vi "Define_Indicies_Connect_Points_Subtracks-1.vi"(3 "error IN":errorcluster, 4 "[IN] Index of track with\n(problem displacement)":i32, 5 "[IN] Index of problem\ndisplacement inside track":i32, 6 "[IN] Track group":T1) -> (0 "error OUT":errorcluster, 1 "[OUT] Index of \nconnected dots\ninside the track":i32[](array[numeric]), 2 "[OUT] Index of connected\ntracks with problem dot":i32[](array[numeric]))   [LabVIEW 2017]
doc: "The subVI scans subtracks for defining connected with input problem point"
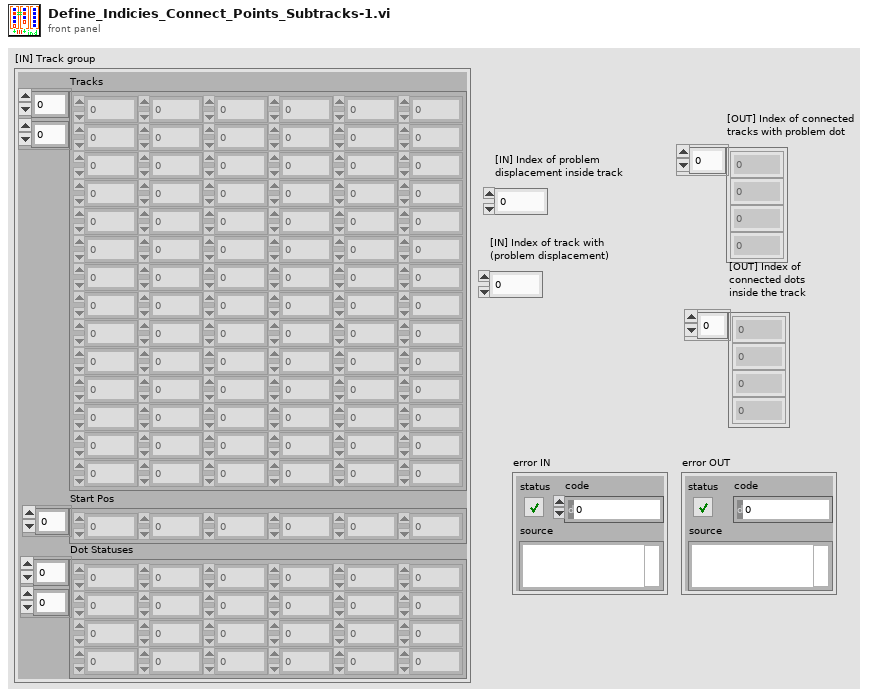
[diagram p1: front panel]
types:
  T1 = cluster{"Tracks":dbl[][], "Start Pos":i32[], "Dot Statuses":i16[][]}
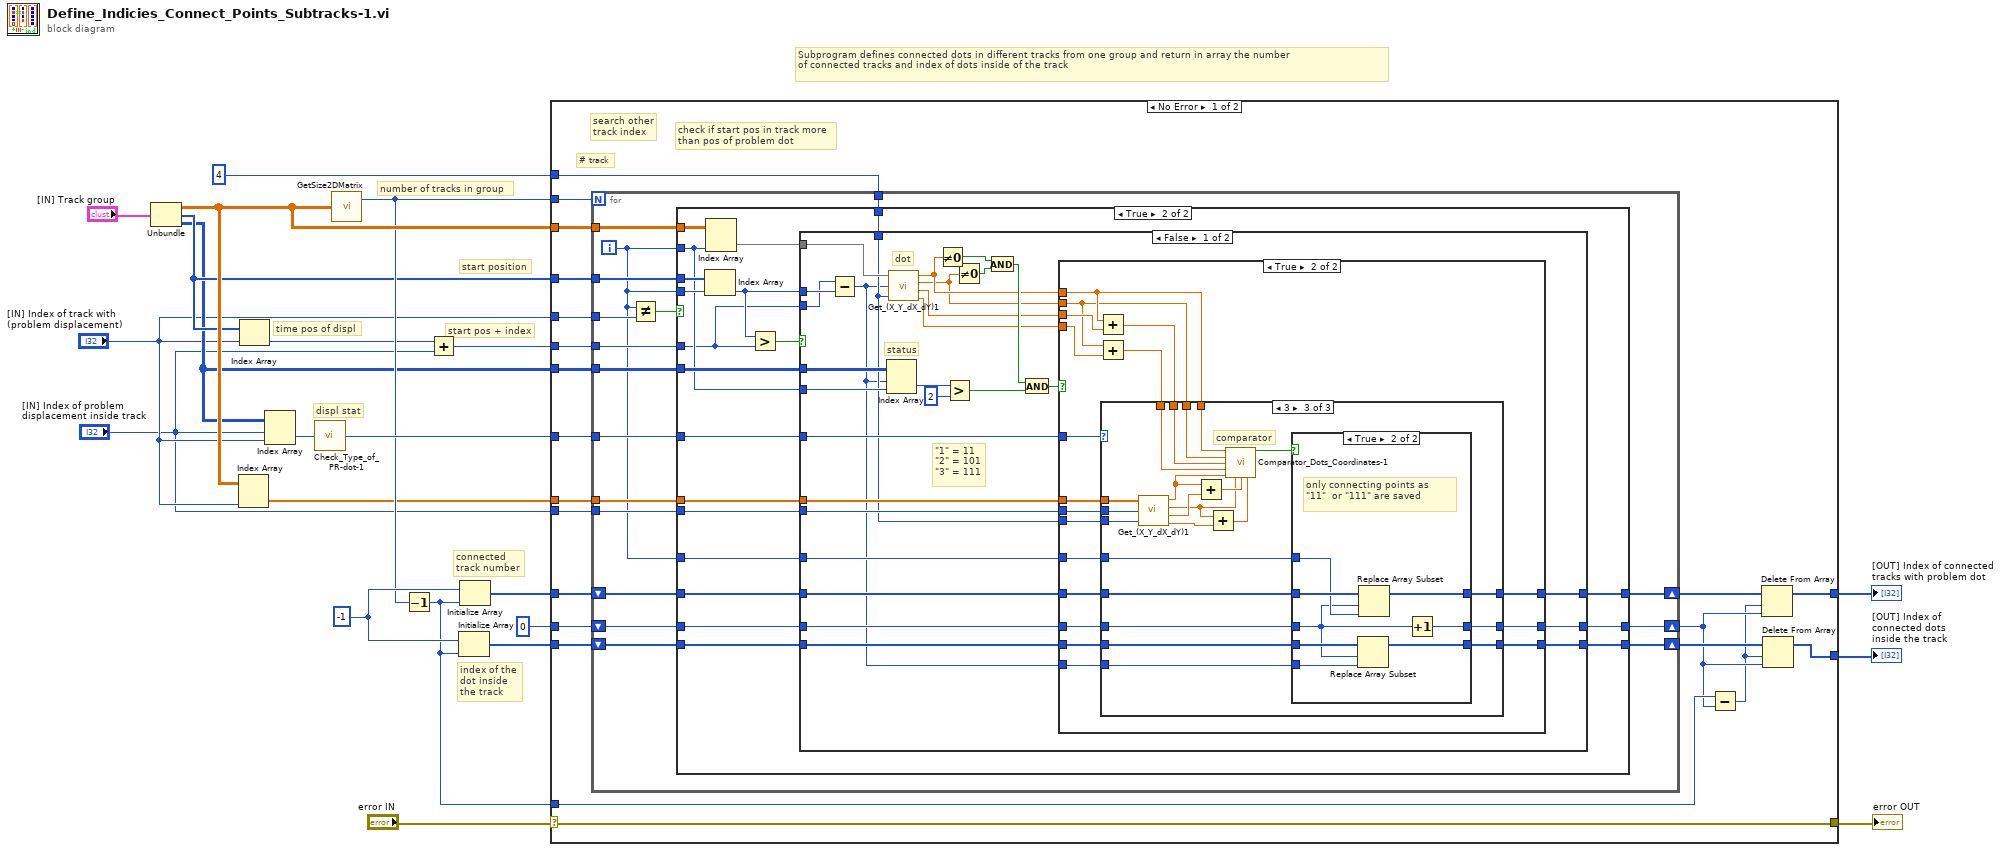
[diagram p0: block diagram]
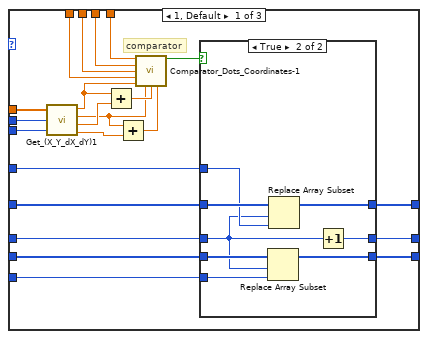
[diagram p4: hidden frame]
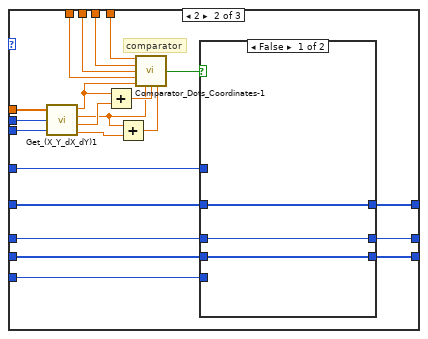
[diagram p6: hidden frame]
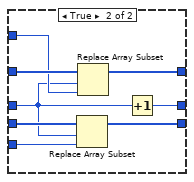
[diagram p7: hidden frame]
diagram:
  w18 = -1 ("disabled index (row)")
  # "start pos + index"
  # "Subprogram defines connected dots in different tracks from one group and return in array the number\nof connected tracks and index of dots inside of the track"
  # "start position"
  # "number of tracks in group"
  # "time pos of displ"
  # "index of the dot inside \nthe track"
  # "connected\ntrack number"
  # "displ stat"
  n1 = Unbundle("[IN] Track group") -> ("Tracks"=w20:dbl[][], "Start Pos"=w13:i32[], "Dot Statuses"=w11:i16[][])
  n2 = Index Array(array=w20, index (col)="[IN] Index of track with\n(problem displacement)") -> (element=w10:dbl[])  [unwired: 1 in]
  n3 = Index Array(array=w13, index="[IN] Index of track with\n(problem displacement)") -> (element=w4:i32)
  n4 = Index Array(array=w11, index (row)="[IN] Index of problem\ndisplacement inside track", index (col)="[IN] Index of track with\n(problem displacement)") -> (element=w21:i16)
  n5 = call "Check_Type_of_PR-dot-1.vi"("[IN] dot status"=w21) -> ("[OUT] Type of\nproblem dot"=w19:i32)
  n6 = call "GetSize2DMatrix.vi"("Array IN (2D)"=w20) -> ("# Cols"=w17:i32)  [unwired: 1 out]
  n7 = Decrement(x=w17) -> (x-1=w9:i32)
  n8 = Add(x=w4, y="[IN] Index of problem\ndisplacement inside track") -> (x+y=w6:i32)
  n9 = Initialize Array(w18, w9) -> (w15:i32[])
  n10 = Initialize Array(w18, w9) -> (w16:i32[])
  n11 = case shown="No Error" "error IN" {
    selector: "error IN" -> [w23 w235]
    tunnel: w20 -> [w43 _]
    tunnel: w19 -> [w42 _]
    tunnel: w17 -> [w41 _]
    tunnel: w16 -> [w40 w237]
    tunnel: w15 -> [w39 w236]
    tunnel: 0 -> [w38 _]
    tunnel: w13 -> [w37 _]
    tunnel: 4 ("multiplier") -> [w36 _]
    tunnel: w11 -> [w35 _]
    tunnel: w10 -> [w34 _]
    tunnel: w9 -> [w32 _]
    tunnel: [w28 w237] -> w8
    tunnel: [w27 w236] -> w7
    tunnel: w6 -> [w26 _]
    tunnel: "[IN] Index of track with\n(problem displacement)" -> [w25 _]
    tunnel: "[IN] Index of problem\ndisplacement inside track" -> [w24 _]
    tunnel: [w23 w235] -> w1
    frame No Error {
      # "# track"
      # "check if start pos in track more \nthan pos of problem dot"
      # "search other\ntrack index"
      n12 = for {
        N: w41 -> [_]
        tunnel: w43 -> [w58]
        tunnel: w42 -> [w54]
        tunnel: w26 -> [w55]
        shift-right: [w46] -> w33
        shift-left: w40 -> [w57]
        shift-right: [w44] -> w31
        shift-left: w39 -> [w56]
        tunnel: w25 -> [w60]
        shift-right: [w45] -> w30
        shift-left: w38 -> [w53]
        tunnel: w37 -> [w52]
        tunnel: w36 -> [w51]
        tunnel: w35 -> [w50]
        tunnel: w34 -> [w49]
        tunnel: w24 -> [w48]
        i -> [w47]
        n13 = Not Equal?(x=w47, y=w60) -> (x != y?=w59:bool)
        n14 = case shown="True" w59 {
          tunnel: w58 -> [_ w83]
          tunnel: w47 -> [_ w75]
          tunnel: w57 -> [w63 w71]
          tunnel: w56 -> [w61 w69]
          tunnel: w55 -> [_ w64]
          tunnel: w54 -> [_ w74]
          tunnel: w53 -> [w62 w70]
          tunnel: w52 -> [_ w82]
          tunnel: w47 -> [_ w81]
          tunnel: w51 -> [_ w77]
          tunnel: w50 -> [_ w76]
          tunnel: w49 -> [_ w73]
          tunnel: w48 -> [_ w72]
          tunnel: w47 -> [_ w68]
          tunnel: [w63 w67] -> w46
          tunnel: [w62 w66] -> w45
          tunnel: [w61 w65] -> w44
          frame False {
          }
          frame True {
            n15 = Index Array(array=w82, index=w81) -> (element=w78:i32)
            n16 = Index Array(array=w83, index (col)=w75) -> (element=w79:dbl[])  [unwired: 1 in]
            n17 = Greater?(x=w78, y=w64) -> (0:w80:bool)
            n18 = case shown="False" w80 {
              tunnel: w79 -> [w111 _]
              tunnel: w78 -> [w110 _]
              tunnel: w64 -> [w109 _]
              tunnel: w77 -> [w92 _]
              tunnel: w76 -> [w106 _]
              tunnel: w75 -> [w105 _]
              tunnel: w74 -> [w99 _]
              tunnel: w73 -> [w94 _]
              tunnel: w72 -> [w93 _]
              tunnel: w71 -> [w91 w234]
              tunnel: w70 -> [w90 w233]
              tunnel: w69 -> [w89 w232]
              tunnel: w68 -> [w88 _]
              tunnel: [w86 w234] -> w67
              tunnel: [w85 w233] -> w66
              tunnel: [w84 w232] -> w65
              frame False {
                # "\"1\" = 11\n\"2\" = 101\n\"3\" = 111"
                # "status"
                # "dot"
                n19 = Subtract(x=w109, y=w110) -> (x-y=w87:i32)
                n20 = Index Array(array=w106, index (row)=w87, index (col)=w105) -> (element=w104:i16)
                n21 = call "Get_(X_Y_dX_dY)1.vi"("(X,Y,dX,dY)"=w111, "index"=w87, "multiplier"=w92) -> ("X"=w98:dbl, "Y"=w97:dbl, "dX"=w96:dbl, "dY"=w95:dbl)
                n22 = Not Equal To 0?(x=w98) -> (x != 0?=w107:bool)
                n23 = Greater?(x=w104, y=i16 2) -> (0:w101:bool)
                n24 = Not Equal To 0?(x=w97) -> (x != 0?=w108:bool)
                n25 = And(x=w107, y=w108) -> (x .and. y?=w102:bool)
                n26 = And(x=w102, y=w101) -> (x .and. y?=w100:bool)
                n27 = case shown="True" w100 {
                  tunnel: w99 -> [_ w132]
                  tunnel: w98 -> [_ w126]
                  tunnel: w97 -> [_ w125]
                  tunnel: w96 -> [_ w128]
                  tunnel: w95 -> [_ w127]
                  tunnel: w94 -> [_ w131]
                  tunnel: w93 -> [_ w130]
                  tunnel: w92 -> [_ w129]
                  tunnel: w91 -> [w114 w122]
                  tunnel: w90 -> [w113 w121]
                  tunnel: w89 -> [w112 w120]
                  tunnel: w88 -> [_ w119]
                  tunnel: w87 -> [_ w118]
                  tunnel: [w114 w117] -> w86
                  tunnel: [w113 w116] -> w85
                  tunnel: [w112 w115] -> w84
                  frame False {
                  }
                  frame True {
                    n28 = Add(x=w126, y=w128) -> (x+y=w124:dbl)
                    n29 = Add(x=w125, y=w127) -> (x+y=w123:dbl)
                    n30 = case shown="3" w132 {
                      tunnel: w131 -> [w154 w177 w214]
                      tunnel: w130 -> [w153 w176 w213]
                      tunnel: w129 -> [w152 w175 w212]
                      tunnel: w126 -> [w151 w178 w208]
                      tunnel: w125 -> [w150 w179 w209]
                      tunnel: w124 -> [w149 w180 w210]
                      tunnel: w123 -> [w148 w181 w211]
                      tunnel: w122 -> [w140 w172 w206]
                      tunnel: w121 -> [w139 w171 w205]
                      tunnel: w120 -> [w138 w170 w204]
                      tunnel: w119 -> [w137 w173 w207]
                      tunnel: w118 -> [w136 w169 w203]
                      tunnel: [w135 w168 w202] -> w117
                      tunnel: [w134 w167 w201] -> w116
                      tunnel: [w133 w166 w200] -> w115
                      frame 1, Default {
                        # "comparator"
                        n31 = call "Get_(X_Y_dX_dY)1.vi"("(X,Y,dX,dY)"=w154, "index"=w153, "multiplier"=w152) -> ("X"=w147:dbl, "Y"=w144:dbl, "dX"=w146:dbl, "dY"=w143:dbl)
                        n32 = Add(x=w147, y=w146) -> (x+y=w145:dbl)
                        n33 = Add(x=w144, y=w143) -> (x+y=w142:dbl)
                        n34 = call "Comparator_Dots_Coordinates-1.vi"("X1"=w151, "Y1"=w150, "(X+dX)1"=w149, "(Y+dY)1"=w148, "X2"=w147, "Y2"=w144, "(X+dX)2"=w145, "(Y+dY)2"=w142) -> ("X1=X2,Y1=Y2 (1)"=w141:bool)  [unwired: 5 in, 2 out]
                        n35 = case shown="True" w141 {
                          tunnel: w140 -> [w157 w165]
                          tunnel: w139 -> [w156 w161]
                          tunnel: w138 -> [w155 w163]
                          tunnel: w137 -> [_ w164]
                          tunnel: w136 -> [_ w162]
                          tunnel: [w157 w160] -> w135
                          tunnel: [w156 w159] -> w134
                          tunnel: [w155 w158] -> w133
                          frame False {
                          }
                          frame True {
                            n36 = Replace Array Subset(array=w163, new element=w162, index=w161) -> (w158:i32[])
                            n37 = Replace Array Subset(array=w165, new element=w164, index=w161) -> (w160:i32[])
                            n38 = Increment(x=w161) -> (x+1=w159:i32)
                          }
                        }
                      }
                      frame 2 {
                        # "comparator"
                        n39 = call "Get_(X_Y_dX_dY)1.vi"("(X,Y,dX,dY)"=w177, "index"=w176, "multiplier"=w175) -> ("X"=w187:dbl, "Y"=w184:dbl, "dX"=w186:dbl, "dY"=w183:dbl)
                        n40 = Add(x=w187, y=w186) -> (x+y=w185:dbl)
                        n41 = Add(x=w184, y=w183) -> (x+y=w182:dbl)
                        n42 = call "Comparator_Dots_Coordinates-1.vi"("X1"=w178, "Y1"=w179, "(X+dX)1"=w180, "(Y+dY)1"=w181, "X2"=w187, "Y2"=w184, "(X+dX)2"=w185, "(Y+dY)2"=w182) -> ("X1(2)=X2(2),Y1(2)=Y2(2) (2)"=w174:bool)  [unwired: 5 in, 2 out]
                        n43 = case shown="False" w174 {
                          tunnel: w172 -> [w190 w198]
                          tunnel: w171 -> [w189 w194]
                          tunnel: w170 -> [w188 w196]
                          tunnel: w173 -> [_ w197]
                          tunnel: w169 -> [_ w195]
                          tunnel: [w190 w193] -> w168
                          tunnel: [w189 w192] -> w167
                          tunnel: [w188 w191] -> w166
                          frame False {
                          }
                          frame True {
                            n44 = Replace Array Subset(array=w196, new element=w195, index=w194) -> (w191:i32[])
                            n45 = Replace Array Subset(array=w198, new element=w197, index=w194) -> (w193:i32[])
                            n46 = Increment(x=w194) -> (x+1=w192:i32)
                          }
                        }
                      }
                      frame 3 {
                        # "comparator"
                        n47 = call "Get_(X_Y_dX_dY)1.vi"("(X,Y,dX,dY)"=w214, "index"=w213, "multiplier"=w212) -> ("X"=w220:dbl, "Y"=w217:dbl, "dX"=w219:dbl, "dY"=w216:dbl)
                        n48 = Add(x=w220, y=w219) -> (x+y=w218:dbl)
                        n49 = Add(x=w217, y=w216) -> (x+y=w215:dbl)
                        n50 = call "Comparator_Dots_Coordinates-1.vi"("X1"=w208, "Y1"=w209, "(X+dX)1"=w210, "(Y+dY)1"=w211, "X2"=w220, "Y2"=w217, "(X+dX)2"=w218, "(Y+dY)2"=w215) -> ("X1=X2,Y1=Y2 (1)"=w199:bool)  [unwired: 5 in, 2 out]
                        n51 = case shown="True" w199 {
                          tunnel: w206 -> [w223 w231]
                          tunnel: w205 -> [w222 w227]
                          tunnel: w204 -> [w221 w229]
                          tunnel: w207 -> [_ w230]
                          tunnel: w203 -> [_ w228]
                          tunnel: [w223 w226] -> w202
                          tunnel: [w222 w225] -> w201
                          tunnel: [w221 w224] -> w200
                          frame False {
                          }
                          frame True {
                            # "only connecting points as \n\"11\"  or \"111\" are saved"
                            n52 = Replace Array Subset(array=w229, new element=w228, index=w227) -> (w224:i32[])
                            n53 = Replace Array Subset(array=w231, new element=w230, index=w227) -> (w226:i32[])
                            n54 = Increment(x=w227) -> (x+1=w225:i32)
                          }
                        }
                      }
                    }
                  }
                }
              }
              frame True {
              }
            }
          }
        }
      }
      n55 = Subtract(x=w32, y=w30) -> (x-y=w29:i32)
      n56 = Delete From Array(array=w33, length=w29, index=w30) -> (array with subset deleted=w28:i32[])  [unwired: 1 out]
      n57 = Delete From Array(array=w31, length=w29, index=w30) -> (array with subset deleted=w27:i32[])  [unwired: 1 out]
    }
    frame Error {
    }
  }
  "[OUT] Index of connected\ntracks with problem dot" <- w8
  "[OUT] Index of \nconnected dots\ninside the track" <- w7
  "error OUT" <- w1
